vi "Write Relay All Off.vi"(8 "error in (no error)":errorcluster, 11 "Device":string="hidraw0") -> (0 "error out":errorcluster)   [LabVIEW 2021, in "USB Relay Control.lvlib"]
uses:
  typedef/Read Write.ctl
  USB Relay Control.lvlib
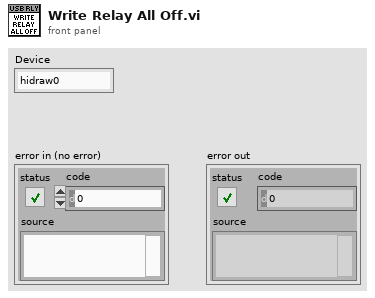
[diagram p1: front panel]
types:
  T1 = typedef "USB Relay Control.lvlib/Read Write.ctl" = enum8{"Read", "Write"}
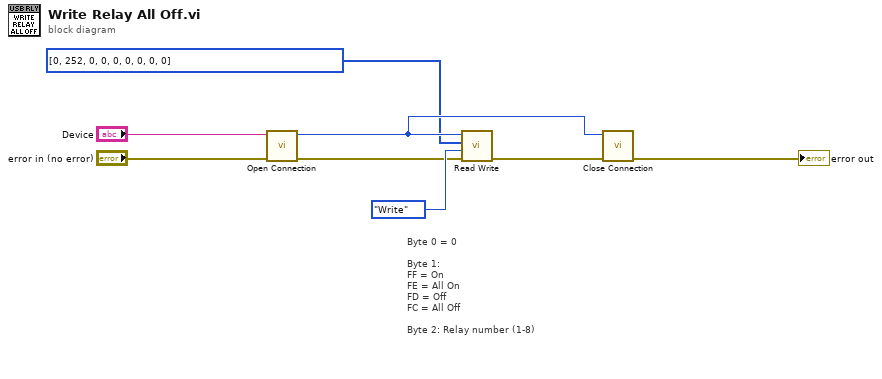
[diagram p0: block diagram]
diagram:
  # "Byte 0 = 0\n\nByte 1:\nFF = On\nFE = All On\nFD = Off\nFC = All Off\n\nByte 2: Relay number (1-8)"
  n1 = call "Open Connection.vi"("error in (no error)"="error in (no error)", "Device"="Device") -> ("error out"=w5:errorcluster, "HID RAW Reference"=w7:i32)  [unwired: 8 in]
  n2 = call "Read Write.vi"("error in (no error)"=w5, "RW"=Read_Write."Write", "Buffer In"=u8[] [0, 252, 0, 0, 0, 0, 0, 0, 0], "HID RAW Reference"=w7) -> ("error out"=w2:errorcluster)  [unwired: 6 in, 1 out]
  n3 = call "Close Connection.vi"("error in (no error)"=w2, "HID RAW Reference"=w7) -> ("error out"=→"error out":errorcluster)  [unwired: 9 in]
